vi "ZL300 Stage Engine.vi"(0 "Notifier Name":string="Not a Name", 11 "Unused Array":string[](array[string])) -> ()   [LabVIEW 2016]
uses:
  Stages Controls/Stage Focus Control.ctl
  Stages Controls/Stage Status.ctl
  Stages Controls/Stage Notifier Element.ctl
  Stages Controls/Stage Actions.ctl
  MCL Libraries/Madlib.dll
panel:
  out "Status":T1
  in  "QUIT":bool
  in  "Focus Control":T2
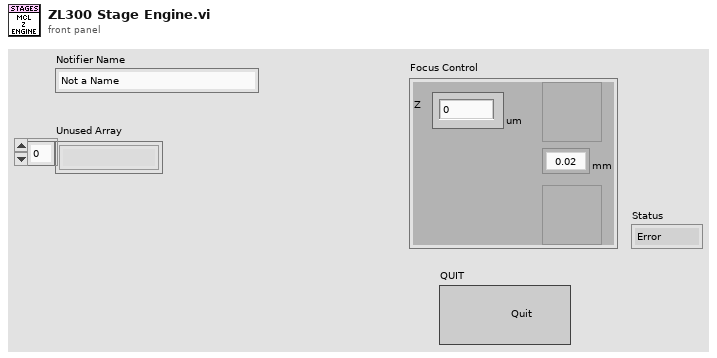
[diagram p1: front panel]
types:
  T1 = typedef "Stage Status.ctl" = enum16{"Error", "Abort", "Busy", "On Target"}
  T2 = typedef "Stage Focus Control.ctl" = cluster{"Focus Step (um)":enum16{"0.02", "0.05", "0.1", "0.5", "1", "2", "5", "10", "20"}, "Focus Up":bool, "Focus Down":bool, "Z ":dbl}
  T3 = typedef "Stage Notifier Element.ctl" = cluster{"Action":T4, "Axis":bool[], "Setpoint":dbl[], "Velocity":dbl, "Cmd Recvd?":bool, "Position":dbl[], "Status":T1, "Misc":variant}
  T4 = typedef "Stage Actions.ctl" = enum16{"Get Position", "MVR", "MOVE", "HALT", "ONTARGET", "ERROR", "REFERENCE", "INIT", "VELOCITY", "STATUS", "EXIT", "HOME", "ZEROPOS", "NANOPOS", "ANALOG", "QUIT"}
  T5 = enum32{"Invalid", "Standard", "Closed", "Hidden", "Minimized", "Maximized"}
  T6 = cluster{"Focus Step (um)":bool, "Focus Up":bool, "Focus Down":bool, "Z ":bool}
  T7 = enum16{"0.02", "0.05", "0.1", "0.5", "1", "2", "5", "10", "20"}
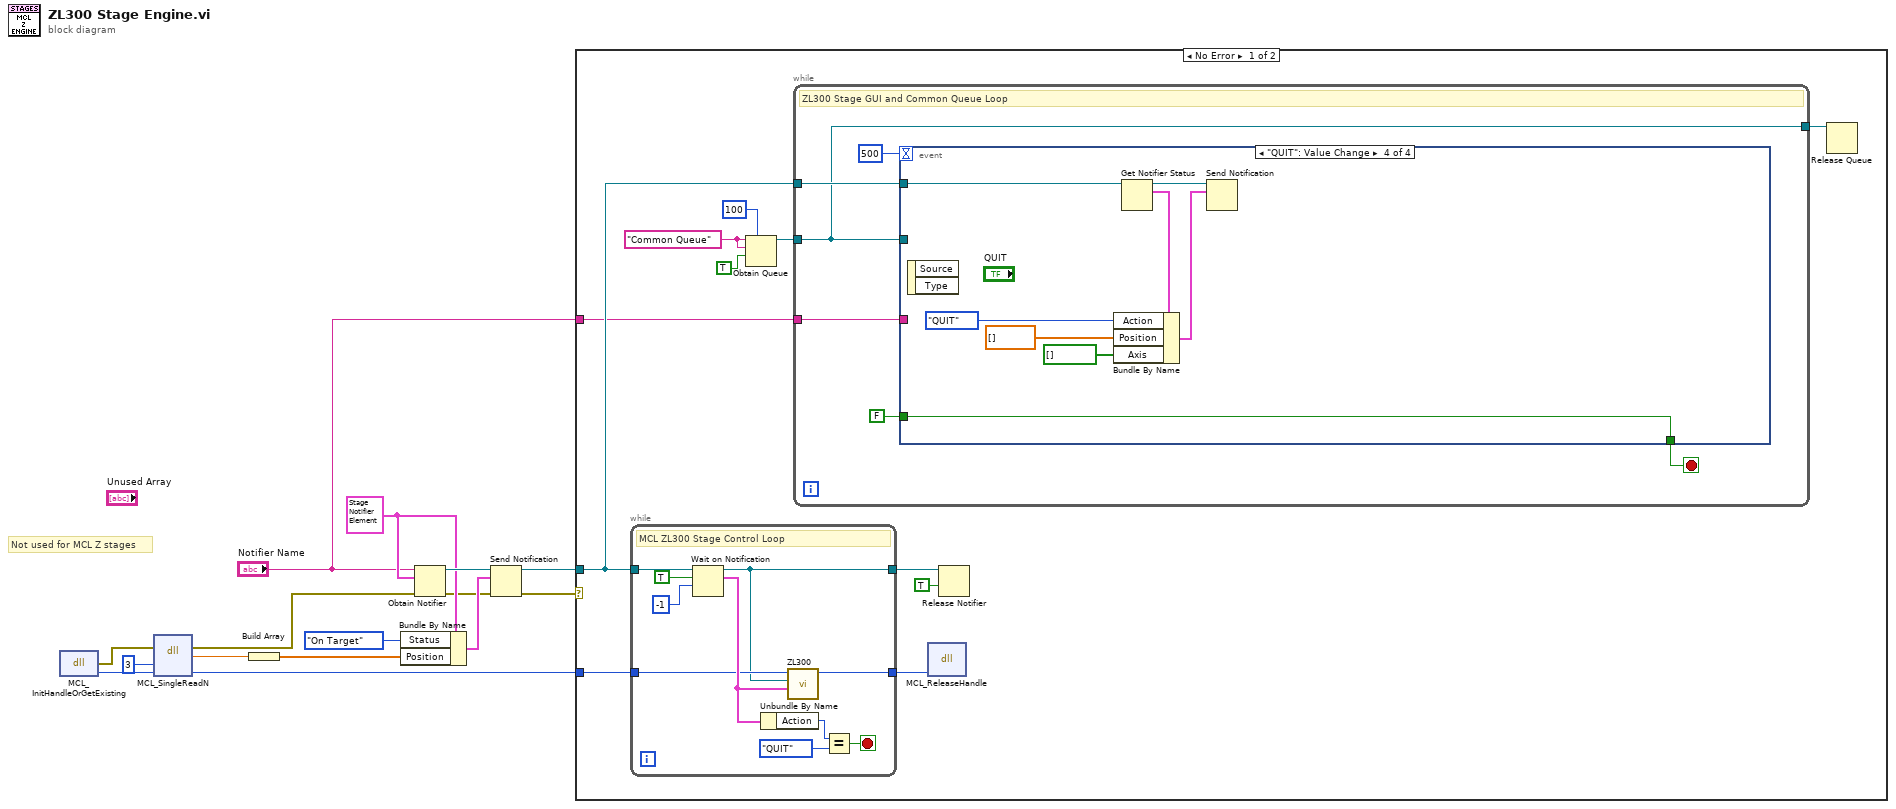
[diagram p0: block diagram]
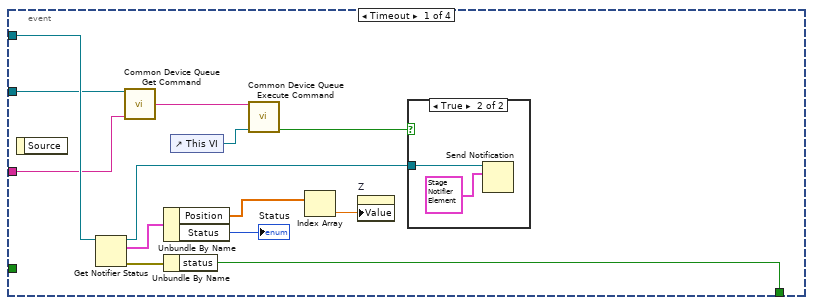
[diagram p2: hidden frame]
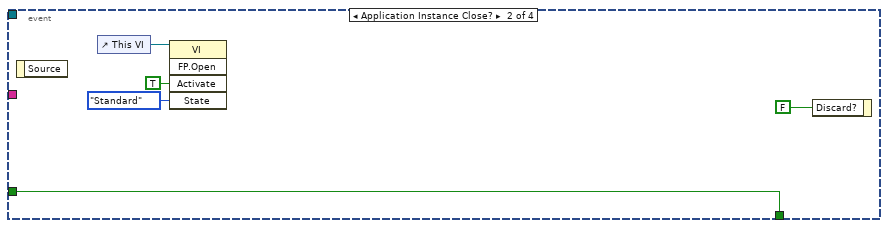
[diagram p4: hidden frame]
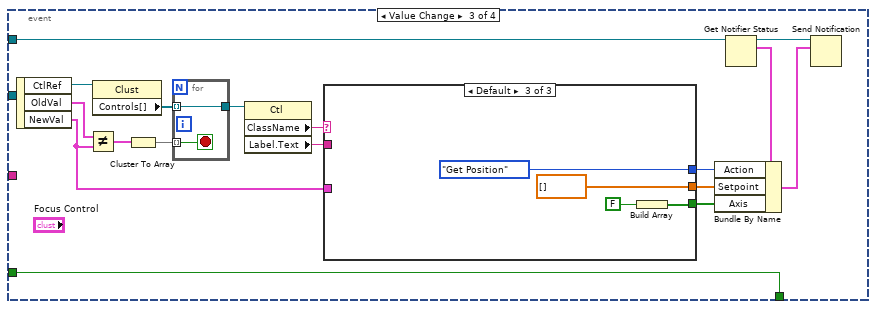
[diagram p5: hidden frame]
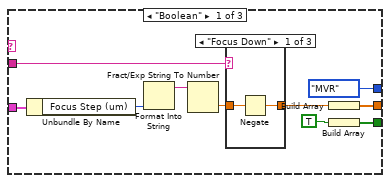
[diagram p6: hidden frame]
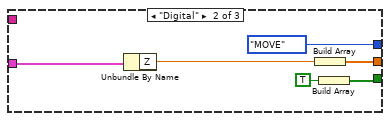
[diagram p9: hidden frame]
diagram:
  w11 = T3 {"Action"=enum."Get Position", "Axis"=[], "Setpoint"=[], "Velocity"=0.5, "Cmd Recvd?"=FALSE, "Position"=[], "Status"=enum."Abort", "Misc"=variant} ("Stage Status")
  # "Not used for MCL Z stages"
  n1 = dll-call lib="C:/Users/4PiSMS/Documents/Microscope-Control/Device Library/Stages/Mad City Labs/ZL300/MCL Libraries/MADLib.dll" fn="MCL_InitHandleOrGetExisting"() -> (error out=w5:errorcluster, w6:i32)  [unwired: 3 in, 1 out]
  n2 = dll-call lib="C:/Users/4PiSMS/Documents/Microscope-Control/Device Library/Stages/Mad City Labs/ZL300/MCL Libraries/MADLib.dll" fn="MCL_SingleReadN"(error in=w5, "axis"=u32 3, "handle"=w6) -> (error out=w4:errorcluster, "return type"=w13:dbl, "handle"=w15:i32)  [unwired: 3 in, 1 out]
  n3 = Build Array(w13) -> (w8:dbl[])
  n4 = Bundle By Name(cluster=w11, "Status"=Stage_Status."On Target", "Position"=w8) -> (w10:T3)
  n5 = Obtain Notifier(name (unnamed)="Notifier Name", notification data type=w11, error in (no error)=w4) -> (notifier out=w12:refnum<notifier>, error out=w3:errorcluster)  [unwired: 1 in, 1 out]
  n6 = Send Notification(notification=w10, notifier=w12, error in (no error)=w3) -> (notifier out=w9:refnum<notifier>, error out=w2:errorcluster)
  n7 = case shown="No Error" w2 {
    tunnel: w15 -> [w26 _]
    tunnel: w9 -> [w24 _]
    tunnel: "Notifier Name" -> [w17 _]
    frame No Error {
      w21 = "Common Queue" ("Unique Notifier Name")
      n8 = while {
        tunnel: w26 -> [w33]
        tunnel: [w35] -> w22
        tunnel: w24 -> [w30]
        tunnel: [w32] -> w23
        stop <- w34 stop-if-true
        # "MCL ZL300 Stage Control Loop"
        n9 = Wait on Notification(notifier=w30, ignore previous (F)=TRUE, timeout in ms (-1)=-1) -> (notifier out=w32:refnum<notifier>, notification=w36:T3)  [unwired: 1 in, 2 out]
        n10 = Unbundle By Name(w36) -> ("Action"=w28:T4)
        n11 = call "ZL300.vi"("Stage Action"=w36, "Stage Status"=w32, "MCL Handle"=w33) -> ("handle out"=w35:i32)  [unwired: 8 in]
        n12 = Equal?(x=w28, y=Stage_Actions."QUIT") -> (x = y?=w34:bool)
      }
      n13 = Obtain Queue(max queue size (-1, unlimited)=100, name (unnamed)=w21, element data type=w21, create if not found? (T)=TRUE) -> (queue out=w18:refnum<queue>)  [unwired: 1 in, 2 out]
      n14 = while {
        tunnel: w24 -> [w40]
        tunnel: w18 -> [w37]
        tunnel: w17 -> [w38]
        tunnel: [w37] -> w16
        stop <- w41 stop-if-true
        # "ZL300 Stage GUI and Common Queue Loop"
        n15 = event shown="[3] \"QUIT\": Value Change" {
          selector: _ -> [_ _ _ _]
          dyn-events: _ -> [_ _ _ _]
          timeout: 500 -> [_ _ _ _]
          tunnel: [w55 w58 w63 w106] -> w41
          tunnel: w40 -> [w53 _ w68 w110]
          tunnel: FALSE ("status") -> [_ w58 w63 w106]
          tunnel: w37 -> [w45 _ _ _]
          tunnel: w38 -> [w43 _ _ _]
          event Timeout {
            n16 = event-data() -> ()  [unwired: 1 in, 1 out]
            n17 = Get Notifier Status(notifier=w53) -> (notifier out=w44:refnum<notifier>, current notification=w52:T3, error out=w50:errorcluster)  [unwired: 1 in, 2 out]
            n18 = call "Common Device Queue Get Command.vi"("Common Queue"=w45, "Notifier Name"=w43) -> ("Command"=w46:string)  [unwired: 12 in, 1 out]
            n19 = Unbundle By Name(w52) -> ("Position"=w51:dbl[], "Status"=→"Status":T1)
            n20 = Unbundle By Name(w50) -> ("status"=w55:bool)
            n21 = control-ref of="This VI"() -> (w47:refnum<vi>)
            n22 = call "Common Device Queue Execute Command.vi"("Common Command"=w46, "VI Refnum"=w47) -> ("Quit?"=w48:bool)  [unwired: 12 in, 1 out]
            n23 = Index Array(array=w51) -> (element=w54:dbl)  [unwired: 1 in]
            n24 = property on="Z" class="DigNum (strict)"("Value"=w54) -> ()  [unwired: 2 in, 2 out]
            n25 = case shown="True" w48 {
              tunnel: w44 -> [_ w57]
              frame False {
              }
              frame True {
                n26 = Send Notification(notification=T3 {"Action"=enum."QUIT", "Axis"=[], "Setpoint"=[], "Velocity"=0.5, "Cmd Recvd?"=FALSE, "Position"=[], "Status"=enum."Error", "Misc"=variant} ("Stage Status"), notifier=w57) -> ()  [unwired: 1 in, 2 out]
              }
            }
          }
          event Application Instance Close? {
            n27 = event-data() -> ()  [unwired: 1 in, 1 out]
            n28 = control-ref of="This VI"() -> (w60:refnum<vi>)
            n29 = invoke class="VI" method="FP.Open"(reference=w60, "Activate"=TRUE ("Activate?"), "State"=T5."Standard") -> ()  [unwired: 2 in, 5 out]
            n30 = event-data("Discard?"=FALSE) -> ()  [unwired: 1 in, 1 out]
          }
          event Value Change {
            n31 = event-data() -> ("CtlRef"=w78:refnum<vi>, "OldVal"=w79:T2, "NewVal"=w72:T2)  [unwired: 1 in]
            n32 = Not Equal?(x=w79, y=w72) -> (x != y?=w77:T6)
            n33 = property class="Clust"(reference=w78) -> ("Controls[]"=w75:refnum<vi>[])  [unwired: 1 in, 2 out]
            n34 = Cluster To Array(cluster=w77) -> (array=w76:bool[])
            n35 = for {
              tunnel: w76 -> [w105] mode=indexing
              tunnel: [w104] -> w74
              tunnel: w75 -> [w104] mode=indexing
              stop <- w105 stop-if-true
            }
            n36 = property class="Ctl"(reference=w74) -> ("ClassName"=w73:string, "Label.Text"=w71:string)  [unwired: 1 in, 2 out]
            n37 = case shown="Default" w73 {
              tunnel: w72 -> [w87 w99 _]
              tunnel: w71 -> [w88 _ _]
              tunnel: [w82 w97 dbl[] []] -> w70
              tunnel: [w81 w96 w102] -> w69
              tunnel: [Stage_Actions."MVR" ("Action") Stage_Actions."MOVE" ("Action") Stage_Actions."Get Position" ("Action")] -> w67
              frame "Boolean" {
                n38 = Unbundle By Name(w87) -> ("Focus Step (um)"=w85:T7)
                n39 = Format Into String(w85) -> (resulting string=w86:string)  [unwired: 3 in, 1 out]
                n40 = Fract/Exp String To Number(string=w86) -> (number=w84:dbl)  [unwired: 3 in, 1 out]
                n41 = case shown="\"Focus Down\"" w88 {
                  tunnel: w84 -> [w91 w92 w93]
                  tunnel: [w90 w92 w93] -> w83
                  frame "Focus Down" {
                    n42 = Negate(x=w91) -> (-x=w90:dbl)
                  }
                  frame "Focus Up" {
                  }
                  frame Default {
                  }
                }
                n43 = Build Array(w83) -> (w82:dbl[])
                n44 = Build Array(TRUE) -> (w81:bool[])
              }
              frame "Digital" {
                n45 = Unbundle By Name(w99) -> ("Z"=w98:dbl)
                n46 = Build Array(w98) -> (w97:dbl[])
                n47 = Build Array(TRUE) -> (w96:bool[])
              }
              frame Default {
                n48 = Build Array(FALSE) -> (w102:bool[])
              }
            }
            n49 = Get Notifier Status(notifier=w68) -> (notifier out=w66:refnum<notifier>, current notification=w65:T3)  [unwired: 1 in, 3 out]
            n50 = Bundle By Name(cluster=w65, "Action"=w67, "Setpoint"=w70, "Axis"=w69) -> (w64:T3)
            n51 = Send Notification(notification=w64, notifier=w66) -> ()  [unwired: 1 in, 2 out]
          }
          event "QUIT": Value Change {
            n52 = event-data() -> ()  [unwired: 1 in, 2 out]
            n53 = Get Notifier Status(notifier=w110) -> (notifier out=w108:refnum<notifier>, current notification=w107:T3)  [unwired: 1 in, 3 out]
            n54 = Bundle By Name(cluster=w107, "Action"=Stage_Actions."QUIT", "Position"=dbl[] [], "Axis"=bool[] []) -> (w111:T3)
            n55 = Send Notification(notification=w111, notifier=w108) -> ()  [unwired: 1 in, 2 out]
          }
        }
      }
      n56 = dll-call lib="C:/Users/4PiSMS/Documents/Microscope-Control/Device Library/Stages/Mad City Labs/ZL300/MCL Libraries/MADLib.dll" fn="MCL_ReleaseHandle"("handle"=w22) -> ()  [unwired: 5 in, 2 out]
      n57 = Release Notifier(notifier=w23, force destroy? (F)=TRUE) -> ()  [unwired: 1 in, 3 out]
      n58 = Release Queue(queue=w16) -> ()  [unwired: 2 in, 3 out]
    }
    frame Error {
    }
  }
